vi "icons-style.vi"() -> ()   [LabVIEW 2024]
panel:
  in  "Numeric":i32
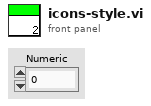
[diagram p1: front panel]
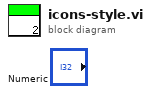
[diagram p0: block diagram]
diagram:
